vi "Read from Data Source.vi"(7 "Project Store in":refnum<class "Project Store.lvclass">, 8 "error in (no error)":errorcluster) -> (0 "error out":errorcluster, 5 "Project Store out":refnum<class "Project Store.lvclass">)   [LabVIEW 2024, in "Project Store.lvclass"]
doc: "Loads the projects and tasks from the data source into the in-memory model. The parent class has no data source and returns the model unchanged; children override it.\n\nGenerated by: Claude"
uses:
  Project Store.lvclass
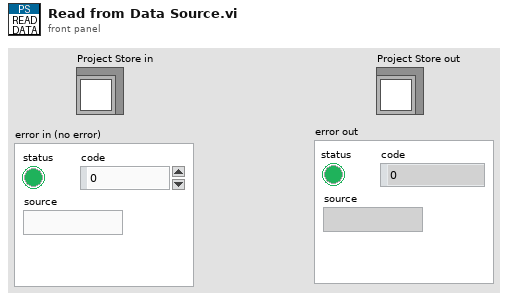
[diagram p1: front panel]
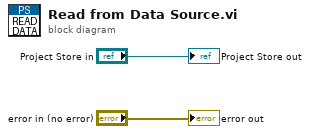
[diagram p0: block diagram]
diagram:
  "Project Store out" <- "Project Store in"
  "error out" <- "error in (no error)"
